vi "Initialize.vi"(6 "node address":u8, 7 "timeout, ms (1000)":u32=1000, 8 "error in (no error)":errorcluster, 10 "baud rate (38400)":u32(ring)=38400 items=["9600"=9600, "19200"=19200, "38400"=38400, "57600"=57600, "115200"=115200, "230400"=230400, "460800"=460800], 11 "port":refnum<visa-resource-name>) -> (0 "error out":errorcluster, 3 "ProPar out":refnum<class "PL Bronkhorst ProPar.lvclass">)   [LabVIEW 2015, in "PL Bronkhorst ProPar.lvclass"]
doc: "Initializes connection to device using specified settings. For single node access <b>node address</b> can be specified once upon initialization. For multiple node access addresses should be specified for each command."
uses:
  PL Bronkhorst ProPar.lvclass
  PL Bronkhorst ProPar.lvclass/PL Bronkhorst ProPar.ctl
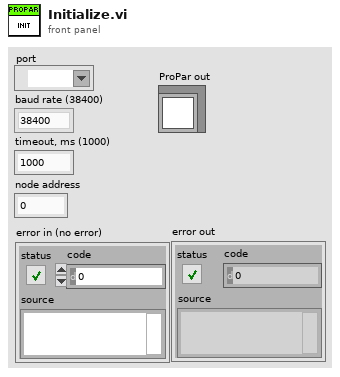
[diagram p1: front panel]
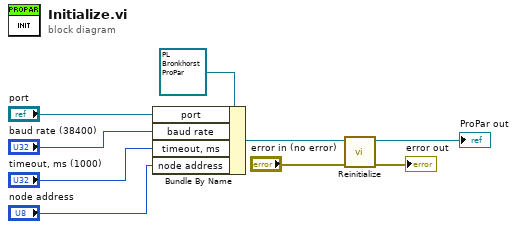
[diagram p0: block diagram]
diagram:
  n1 = Bundle By Name(cluster=refnum<class "PL Bronkhorst ProPar.lvclass"> refnum ("PL Comdel CX.lvclass"), "port"="port", "baud rate"="baud rate (38400)", "timeout, ms"="timeout, ms (1000)", "node address"="node address") -> (w9:refnum<class "PL Bronkhorst ProPar.lvclass">)
  n2 = call "Reinitialize.vi"("error in (no error)"="error in (no error)", "ProPar in"=w9) -> ("error out"=→"error out":errorcluster, "ProPar out"=→"ProPar out":refnum<class "PL Bronkhorst ProPar.lvclass">)  [unwired: 8 in]
